vi "Refresh_List.vi"(8 "error in (no error)":errorcluster, 11 "path":path) -> (0 "error out":errorcluster, 3 "reversed array":string[](array[string]))   [LabVIEW 2025]
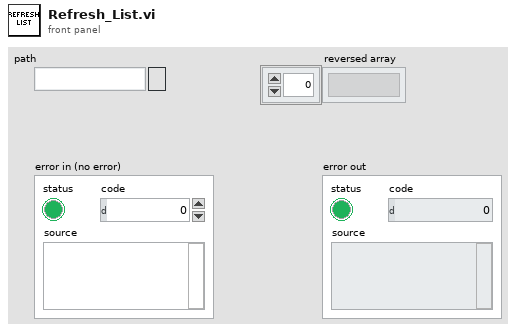
[diagram p1: front panel]
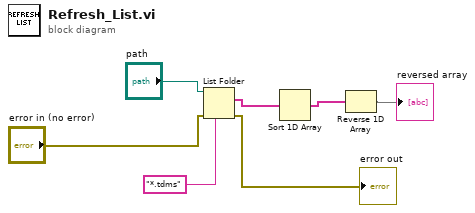
[diagram p0: block diagram]
diagram:
  n1 = List Folder(path="path", pattern="*.tdms", error in="error in (no error)") -> (filenames=w4:string[], error out=→"error out":errorcluster)  [unwired: 1 in, 2 out]
  n2 = Sort 1D Array(array=w4) -> (sorted array=w5:string[])
  n3 = Reverse 1D Array(array=w5) -> (reversed array=→"reversed array":string[])
